vi "Memory Manager Pre-Build.vi"   [LabVIEW 2017]
uses:
  Build Automation.lvlib
types:
  T1 = cluster{"Status Message":refnum<data-value>, "Progress":refnum<data-value>, "Stop":refnum<data-value>}
  T2 = enum16{"Share clones between instances", "Preallocate clone for each instance"}
  T3 = enum32{"invalid VI type", "Standard VI", "Control VI", "Global VI", "Polymorphic VI", "Configuration VI", "SubSystem", "Facade VI", "Method VI", "Statechart Diagram VI"}
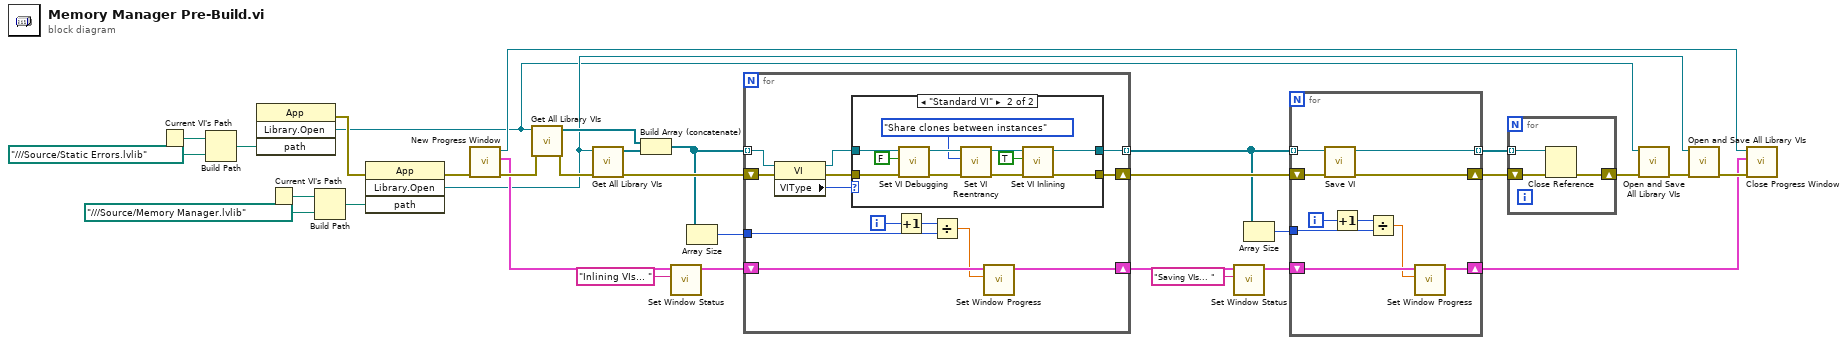
[diagram p0: block diagram]
diagram:
  n1 = Current VI's Path() -> (path=w16:path)
  n2 = Build Path(base path=w16, name or relative path=path "../../../Source/Static Errors.lvlib" ("stripped path")) -> (appended path=w15:path)
  n3 = invoke class="App" method="Library.Open"("path"=w15) -> (error out=w8:errorcluster, "Open Library"=w1:refnum<vi>)  [unwired: 3 in, 2 out]
  n4 = Current VI's Path() -> (path=w21:path)
  n5 = Build Path(base path=w21, name or relative path=path "../../../Source/Memory Manager.lvlib" ("stripped path")) -> (appended path=w33:path)
  n6 = invoke class="App" method="Library.Open"(error in=w8, "path"=w33) -> (error out=w31:errorcluster, "Open Library"=w4:refnum<vi>)  [unwired: 2 in, 2 out]
  n7 = call "New Progress Window.vi"("error in (no error)"=w31) -> ("error out"=w13:errorcluster, "DVRs"=w7:T1, "VI refnum"=w14:refnum<vi>)  [unwired: 8 in]
  n8 = call "Get All Library VIs.vi"("error in (no error)"=w13, "library ref"=w1) -> ("error out"=w12:errorcluster, "vi refs"=w9:refnum<vi>[])  [unwired: 8 in]
  n9 = call "Get All Library VIs.vi"("error in (no error)"=w12, "library ref"=w4) -> ("error out"=w32:errorcluster, "vi refs"=w11:refnum<vi>[])  [unwired: 8 in]
  n10 = Build Array (concatenate)(w9, w11) -> (w10:refnum<vi>[])
  n11 = call "Set Window Status.vi"("Status Message"="Inlining VIs... " ("data value"), "DVRs in"=w7) -> ("DVRs out"=w28:T1)  [unwired: 8 in, 1 out]
  n12 = Array Size(array=w10) -> (size(s)=w29:i32)
  n13 = for {
    tunnel: w10 -> [w39] mode=indexing
    shift-right: [w40] -> w27
    shift-left: w32 -> [w38]
    tunnel: w29 -> [w37]
    shift-right: [w42] -> w26
    shift-left: w28 -> [w44]
    tunnel: [w41] -> w23 mode=indexing
    i -> [w46]
    n14 = property class="VI"(reference=w39, error in=w38) -> (reference out=w36:refnum<vi>, error out=w35:errorcluster, "VIType"=w34:T3)
    n15 = case shown="\"Standard VI\"" w34 {
      tunnel: [w47 w52] -> w41
      tunnel: [w48 w49] -> w40
      tunnel: w35 -> [w48 w51]
      tunnel: w36 -> [w47 w50]
      frame Default {
      }
      frame "Standard VI" {
        n16 = call "Set VI Debugging.vi"("error in (no error)"=w51, "Allow Debugging"=FALSE, "vi ref in"=w50) -> ("error out"=w57:errorcluster, "vi ref out"=w58:refnum<vi>)  [unwired: 7 in]
        n17 = call "Set VI Reentrancy.vi"("error in (no error)"=w57, "Reentrancy Type"=T2."Share clones between instances", "vi ref in"=w58) -> ("error out"=w55:errorcluster, "vi ref out"=w56:refnum<vi>)  [unwired: 7 in]
        n18 = call "Set VI Inlining.vi"("error in (no error)"=w55, "Inline VI"=TRUE, "vi ref in"=w56) -> ("error out"=w49:errorcluster, "vi ref out"=w52:refnum<vi>)  [unwired: 7 in]
      }
    }
    n19 = Increment(x=w46) -> (x+1=w45:i32)
    n20 = Divide(x=w45, y=w37) -> (x/y=w43:dbl)
    n21 = call "Set Window Progress.vi"("Progress"=w43, "DVRs in"=w44) -> ("DVRs out"=w42:T1)  [unwired: 8 in, 1 out]
  }
  n22 = call "Set Window Status.vi"("Status Message"="Saving VIs... ", "DVRs in"=w26) -> ("DVRs out"=w24:T1)  [unwired: 8 in, 1 out]
  n23 = Array Size(array=w23) -> (size(s)=w22:i32)
  n24 = for {
    shift-right: [w67] -> w19
    shift-left: w27 -> [w69]
    tunnel: w23 -> [w68] mode=indexing
    shift-right: [w61] -> w5
    shift-left: w24 -> [w63]
    tunnel: w22 -> [w65]
    tunnel: [w60] -> w18 mode=indexing
    i -> [w64]
    n25 = call "Save VI.vi"("error in (no error)"=w69, "vi ref in"=w68) -> ("error out"=w67:errorcluster, "vi ref out"=w60:refnum<vi>)  [unwired: 8 in]
    n26 = Increment(x=w64) -> (x+1=w66:i32)
    n27 = Divide(x=w66, y=w65) -> (x/y=w62:dbl)
    n28 = call "Set Window Progress.vi"("Progress"=w62, "DVRs in"=w63) -> ("DVRs out"=w61:T1)  [unwired: 8 in, 1 out]
  }
  n29 = for {
    shift-right: [w70] -> w3
    shift-left: w19 -> [w72]
    tunnel: w18 -> [w71] mode=indexing
    n30 = Close Reference(reference=w71, error in (no error)=w72) -> (error out=w70:errorcluster)
  }
  n31 = call "Open and Save All Library VIs.vi"("error in (no error)"=w3, "library ref"=w1) -> ("error out"=w2:errorcluster)  [unwired: 9 in]
  n32 = call "Open and Save All Library VIs.vi"("error in (no error)"=w2, "library ref"=w4) -> ("error out"=w6:errorcluster)  [unwired: 9 in]
  n33 = call "Close Progress Window.vi"("error in (no error)"=w6, "DVRs in"=w5, "VI refnum"=w14) -> ()  [unwired: 8 in, 1 out]
